vi "Release Lock.vi"(8 "error in (no error)":errorcluster, 10 "LockName":string, 11 "Tag in":refnum<class "Tag.lvclass">) -> (0 "error out":errorcluster, 3 "Tag out":refnum<class "Tag.lvclass">)   [LabVIEW 2020, in "Tag Engine Core.lvlib" / "Tag.lvclass"]
doc: "Removes the lock named LockName. Locked becomes FALSE when no locks are left."
uses:
  Tag.lvclass
  Tag.lvclass/Tag.ctl
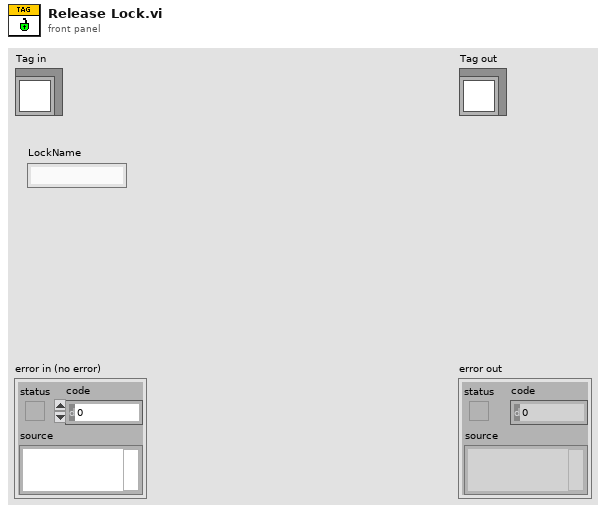
[diagram p1: front panel]
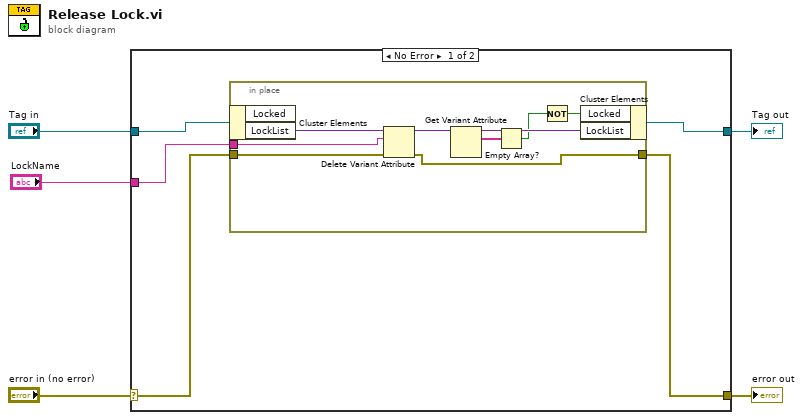
[diagram p0: block diagram]
diagram:
  n1 = case shown="No Error" "error in (no error)" {
    selector: "error in (no error)" -> [w8 w21]
    tunnel: [w7 w21] -> w4
    tunnel: [w9 w20] -> w2
    tunnel: "Tag in" -> [w10 w20]
    tunnel: "LockName" -> [w6 _]
    frame No Error {
      n2 = in-place {
        in-place-border: w8 -> [w17]
        in-place-border: [w11] -> w7
        in-place-border: w6 -> [w18]
        n3 = in-place-cluster #1(w10) -> ("LockList"=w19:variant)  [unwired: 1 out]
        n4 = Delete Variant Attribute(4:w17, 6:w18, 7:w19) -> (0:w11:errorcluster, 3:w16:variant)  [unwired: 1 out]
        n5 = Get Variant Attribute(Variant=w16) -> (duplicate Variant=w14:variant, names=w15:string[])  [unwired: 3 in, 2 out]
        n6 = Empty Array?(array=w15) -> (empty?=w13:bool)
        n7 = Not(x=w13) -> (.not. x?=w12:bool)
        n8 = in-place-cluster #1("Locked"=w12, "LockList"=w14) -> (w9:refnum<class "Tag.lvclass">)
      }
    }
    frame Error {
    }
  }
  "error out" <- w4
  "Tag out" <- w2
